vi "Parse State Queue.vi"(0 "State Queue":string, 7 "Error In (no error)":errorcluster) -> (4 "Remaining States":string, 6 "Current State":string, 8 "Arguments":string)   [LabVIEW 2020]
doc: "Parses the JKI State Machine state queue and returns the current state that will execute next with the associated arguments.\n\nFor instructions on how to use the JKI State Machine, examples and video tutorials, visit:\nhttp://jkisoft.com/state-machine/\n\n<B>Inputs:</B>\n <B>State Queue:</B> The entire state queue is wired to this input. This should come from the main JKI State Machine shift register.\n <B>Error In</B> The error cluster from the JKI State Machine is wired to this input. If an error occures and appears on this input, the current state output returns the \"Error Handler\" state.\n\n<B>Outputs:</B>\n <B>Remaining States:</B> Returns all the next states that should execute after the current state completes. These should be passed through the current state in the state machine. These can also be modified or augmented within the current state if necessary.\n <B>Current State:</B> Returns the current state that should execute next in the state machine. If an error is wired to the Error input then the current state output becomes \"Error Handler\".\n <B>Arguments:</B> Returns any argument(s) that may be used in the current state string. These arguments come after the \">>\" characters. <B>Note:</B> The arguments variable must not contain any unprintable characters like linefeed or carriage return.\n\n<B>State Syntax:</B>\nStateCategory: State >> Argument\nLine Terminator: Line feed\n <B>Example:</B>\nUI: Help >> About\n\nWhere \"UI\" is the state category\nWhere \"Help\" is the state\nWhere \"About\" is the argument\n <B>Other Examples:</B>\nApp Data: Initialize\nUI: Initialize\nHelp >> About\n\n<B>Commenting:</B>\nTo add a comment use \"//\" or \"#\" and all text to the right will be ignored\n <B>Commenting Example:</B>\nUI: Initialize // This initializes the UI\n# This whole line is a comment\n// Another comment line"
panel:
  # "For instructions on how to use the JKI State Machine, examples and video tutorials, visit:\nhttp://jki.net/state-machine/\n\nJKI State Machine™\nhttp://jki.net/state-machine/\nCopyright (C) 2005-2024, JKI <info@jki.net>\nALL RIGHTS RESERVED"
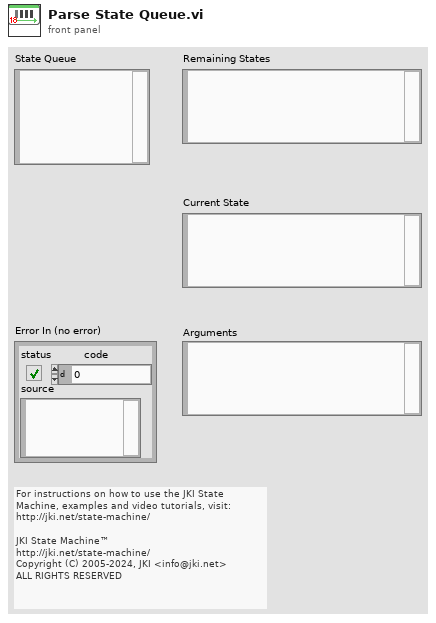
[diagram p1: front panel]
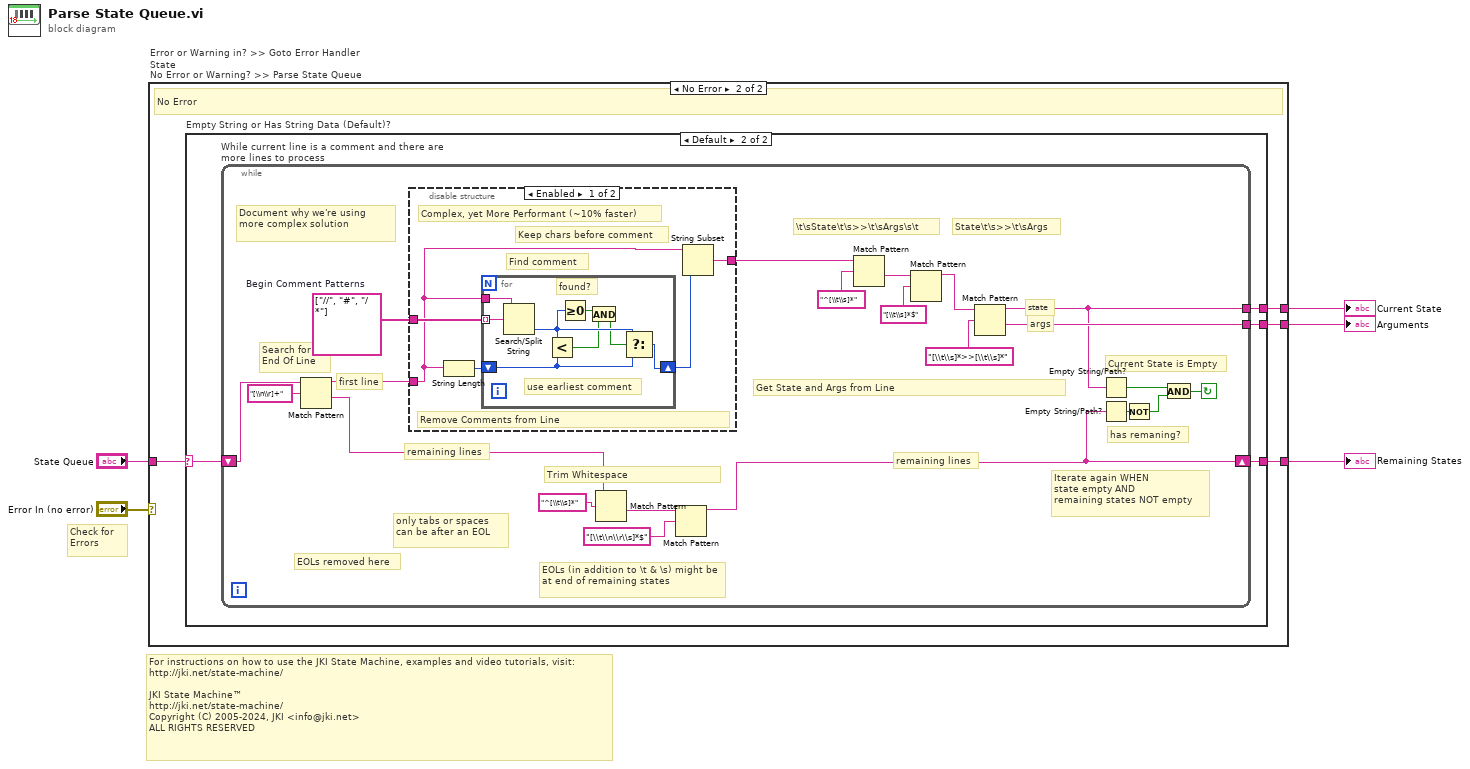
[diagram p0: block diagram]
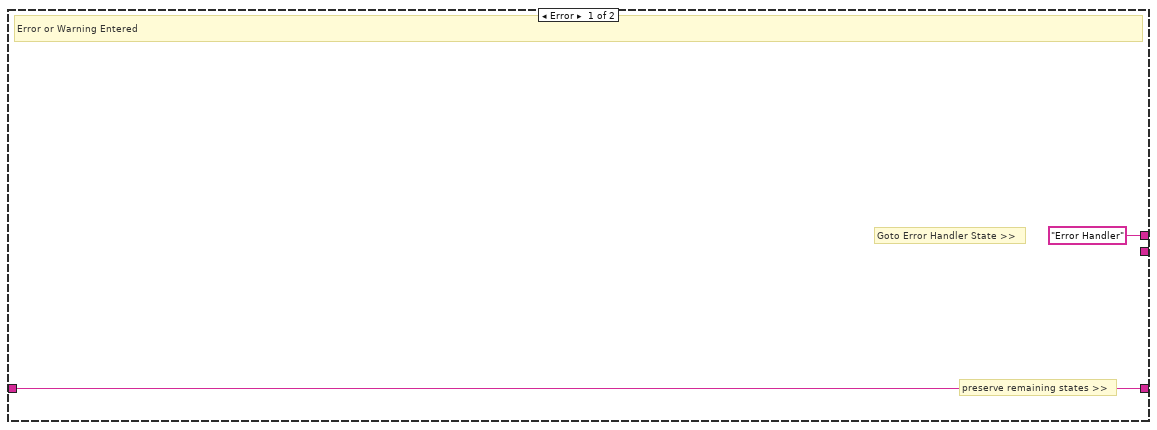
[diagram p2: hidden frame]
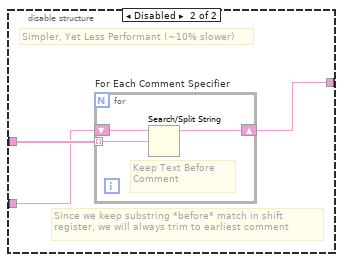
[diagram p4: hidden frame]
diagram:
  # "Check for Errors"
  # "For instructions on how to use the JKI State Machine, examples and video tutorials, visit:\nhttp://jki.net/state-machine/\n\nJKI State Machine™\nhttp://jki.net/state-machine/\nCopyright (C) 2005-2024, JKI <info@jki.net>\nALL RIGHTS RESERVED"
  n1 = case "Error or Warning in? >> Goto Error Handler State\nNo Error or Warning? >> Parse State Queue" shown="No Error" "Error In (no error)" {
    tunnel: [w7 w9] -> w5
    tunnel: ["Error Handler" w11] -> w4
    tunnel: [_ w10] -> w2
    tunnel: "State Queue" -> [w7 w8]
    frame Error {
      # "Goto Error Handler State >>"
      # "preserve remaining states >>"
      # "Error or Warning Entered"
    }
    frame No Error {
      # "No Error"
      n2 = case "Empty String or Has String Data (Default)?" shown="Default" w8 {
        selector: w8 -> [_ w12]
        tunnel: [_ w15] -> w11
        tunnel: [_ w14] -> w10
        tunnel: [_ w13] -> w9
        frame "" {
          # "Do Nothing if Empty String"
          # "<< Wiring into the Case Selector is much more performant than using \"Empty String/Path?\" primitive"
        }
        frame Default {
          n3 = while "While current line is a comment and there are more lines to process" {
            tunnel: [w35] -> w15
            tunnel: [w36] -> w14
            shift-right: [w31] -> w13
            shift-left: w12 -> [w29]
            stop <- w32 continue-if-true
            w28 = string[] ["//", "#", "/*"]  # Begin Comment Patterns
            # "Get State and Args from Line"
            # "State\\t\\s>>\\t\\sArgs"
            # "\\t\\sState\\t\\s>>\\t\\sArgs\\s\\t"
            # "remaining lines"
            # "EOLs (in addition to \\t & \\s) might be at end of remaining states"
            # "Document why we're using more complex solution"
            # "Trim Whitespace"
            # "EOLs removed here"
            # "only tabs or spaces can be after an EOL"
            # "Current State is Empty"
            # "has remaning?"
            # "remaining lines"
            # "first line"
            # "Search for End Of Line"
            # "Iterate again WHEN\nstate empty AND\nremaining states NOT empty"
            # "args"
            # "state"
            n4 = Match Pattern(string=w29, regular expression="[\\n\\r]+") -> (before substring=w27:string, after substring=w19:string)  [unwired: 1 in, 2 out]
            n5 = disable-structure shown="Enabled" {
              disable-tunnel: w28 -> [w41 w52]
              disable-tunnel: [w40 w51] -> w16
              disable-tunnel: w27 -> [w39 w50]
              frame Enabled {
                # "Remove Comments from Line"
                # "Complex, yet More Performant (~10% faster)"
                # "Keep chars before comment"
                # "Find comment"
                n6 = String Length(string=w39) -> (length=w38:i32)
                n7 = for {
                  tunnel: w41 -> [w46] mode=indexing
                  shift-right: [w48] -> w37
                  shift-left: w38 -> [w49]
                  tunnel: w39 -> [w47]
                  # "found?"
                  # "use earliest comment"
                  n8 = Search/Split String(string=w47, search string/char (-)=w46) -> (offset of match=w45:i32)  [unwired: 1 in, 2 out]
                  n9 = Less?(x=w45, y=w49) -> (x < y?=w43:bool)
                  n10 = Greater Or Equal To 0?(x=w45) -> (x >= 0?=w44:bool)
                  n11 = And(x=w44, y=w43) -> (x .and. y?=w42:bool)
                  n12 = Select(t=w45, s=w42, f=w49) -> (s? t:f=w48:i32)
                }
                n13 = String Subset(string=w39, length (rest)=w37) -> (substring=w40:string)  [unwired: 1 in]
              }
              frame Disabled {
                # "Since we keep substring *before* match in shift register, we will always trim to earliest comment"
                # "Simpler, Yet Less Performant (~10% slower)"
                n14 = for "For Each Comment Specifier" {
                  tunnel: w52 -> [w54] mode=indexing
                  shift-right: [w53] -> w51
                  shift-left: w50 -> [w55]
                  # "Keep Text Before Comment"
                  n15 = Search/Split String(string=w55, search string/char (-)=w54) -> (substring before match=w53:string)  [unwired: 1 in, 2 out]
                }
              }
            }
            n16 = Match Pattern(string=w19, regular expression="^[\\t\\s]*") -> (after substring=w18:string)  [unwired: 1 in, 3 out]
            n17 = Match Pattern(string=w18, regular expression="[\\t\\n\\r\\s]*$") -> (before substring=w31:string)  [unwired: 1 in, 3 out]
            n18 = Match Pattern(string=w16, regular expression="^[\\t\\s]*") -> (after substring=w17:string)  [unwired: 1 in, 3 out]
            n19 = Match Pattern(string=w17, regular expression="[\\t\\s]*$") -> (before substring=w21:string)  [unwired: 1 in, 3 out]
            n20 = Match Pattern(string=w21, regular expression="[\\t\\s]*>>[\\t\\s]*") -> (before substring=w35:string, after substring=w36:string)  [unwired: 1 in, 2 out]
            n21 = Empty String/Path?(string/path=w35) -> (empty?=w34:bool)
            n22 = Empty String/Path?(string/path=w31) -> (empty?=w33:bool)
            n23 = Not(x=w33) -> (.not. x?=w26:bool)
            n24 = And(x=w34, y=w26) -> (x .and. y?=w32:bool)
          }
        }
      }
    }
  }
  "Remaining States" <- w5
  "Arguments" <- w2
  "Current State" <- w4
